vi "Test Helper - Echo Server.vi"(6 "Delay 1st reply only":bool, 7 "idle timout":u32=2000, 8 "Answer?":bool, 9 "reply delay (ms)":u32, 10 "number of messages":i32=1, 11 "port":u16=55501) -> (0 "error out":errorcluster, 2 "Commands":string[](array[string]))   [LabVIEW 2019, in "RemoteControl.ZMQ.Tests.lvclass"]
uses:
  RemoteControl.ZMQ.Tests.lvclass
panel:
  out "Numeric":i32
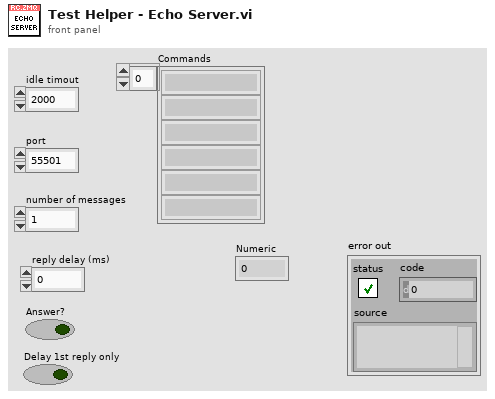
[diagram p1: front panel]
types:
  T1 = typedef "RemoteControl.lvlib/RemoteControl.lvclass/Message--Cluster.ctl" = cluster{"Command":string, "Data":variant, "ID":string, "error":errorcluster}
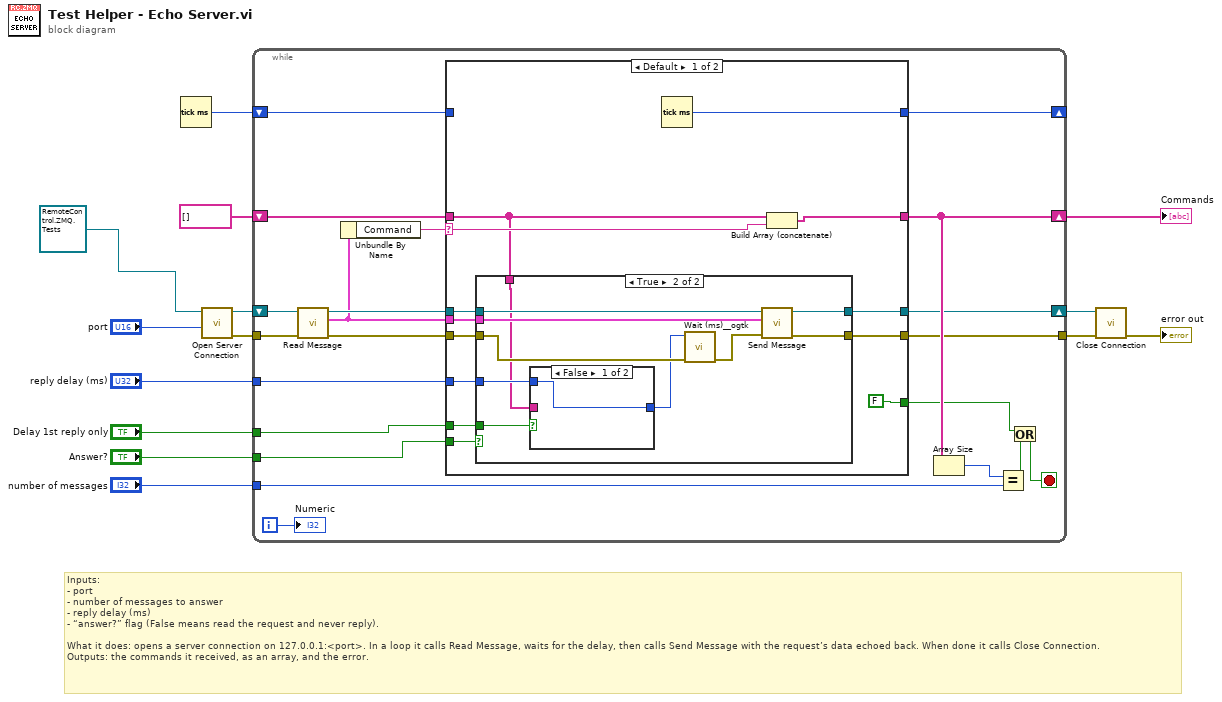
[diagram p0: block diagram]
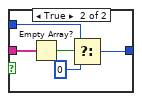
[diagram p3: hidden frame]
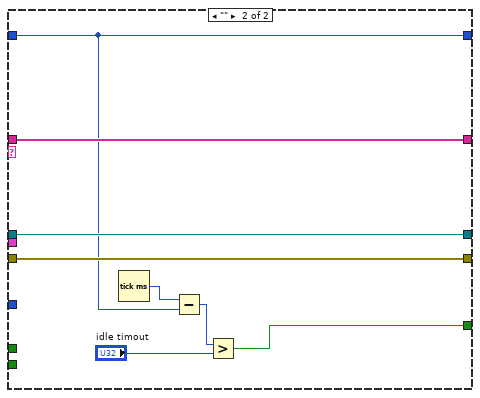
[diagram p4: hidden frame]
diagram:
  # "Inputs:\n- port\n- number of messages to answer\n- reply delay (ms)\n- “answer?” flag (False means read the request and never reply).\n\nWhat it does: opens a server connection on 127.0.0.1:<port>. In a loop it calls Read Message, waits for the delay, then calls Send Message with the request’s data echoed back. When done it calls Close Connection.\nOutputs: the commands it received, as an array, and the error."
  n1 = Tick Count (ms)() -> (millisecond timer value=w2:u32)
  n2 = call-dynamic "Open Server Connection.vi"("port"="port", "RemoteControl.ZMQ in"=refnum<class "RemoteControl.ZMQ.Tests.lvclass"> refnum ("RemoteControl.ZMQ.Tests.lvclass")) -> ("error out"=w12:errorcluster, "RemoteControl.ZMQ out"=w14:refnum<class "RemoteControl.ZMQ.Tests.lvclass">)  [unwired: 8 in]
  n3 = while {
    tunnel: "reply delay (ms)" -> [w18]
    tunnel: w12 -> [w34]
    tunnel: [w25] -> w11
    tunnel: "Answer?" -> [w26]
    tunnel: "number of messages" -> [w33]
    shift-right: [w28] -> w5
    shift-left: string[] [] -> [w30]
    tunnel: "Delay 1st reply only" -> [w19]
    shift-right: [w16] -> _
    shift-left: w2 -> [w15]
    shift-right: [w24] -> w10
    shift-left: w14 -> [w35]
    i -> [w29]
    stop <- w21 stop-if-true
    n4 = call-dynamic "Read Message.vi"("error in (no error)"=w34, "RemoteControl.ZMQ in"=w35) -> ("error out"=w20:errorcluster, "Message"=w17:T1, "RemoteControl.ZMQ out"=w27:refnum<class "RemoteControl.ZMQ.Tests.lvclass">)  [unwired: 7 in]
    n5 = Unbundle By Name(w17) -> ("Command"=w31:string)
    n6 = case shown="Default" w31 {
      selector: w31 -> [w48 _]
      tunnel: [w47 w74] -> w28
      tunnel: w30 -> [w39 w74]
      tunnel: w27 -> [w46 w73]
      tunnel: w26 -> [w45 _]
      tunnel: [w44 w72] -> w25
      tunnel: [w43 w73] -> w24
      tunnel: w17 -> [w42 _]
      tunnel: [FALSE ("x") w67] -> w23
      tunnel: w20 -> [w40 w72]
      tunnel: w19 -> [w38 _]
      tunnel: w18 -> [w37 _]
      tunnel: [w36 w70] -> w16
      tunnel: w15 -> [_ w70]
      frame Default {
        n7 = case shown="True" w45 {
          tunnel: w46 -> [w50 w60]
          tunnel: [w49 w59] -> w44
          tunnel: [w50 w58] -> w43
          tunnel: w42 -> [_ w57]
          tunnel: w40 -> [w49 w55]
          tunnel: w39 -> [_ w52]
          tunnel: w38 -> [_ w51]
          tunnel: w37 -> [_ w54]
          frame False {
          }
          frame True {
            n8 = case shown="False" w51 {
              tunnel: w54 -> [w61 w66]
              tunnel: [w61 w65] -> w53
              tunnel: w52 -> [_ w63]
              frame False {
              }
              frame True {
                n9 = Empty Array?(array=w63) -> (empty?=w62:bool)
                n10 = Select(t=w66, s=w62, f=u32 0) -> (s? t:f=w65:u32)
              }
            }
            n11 = call <userlib>:"Wait (ms)__ogtk.vi"("error in (no error)"=w55, "milliseconds to wait"=w53) -> ("error out"=w56:errorcluster)  [unwired: 8 in, 1 out]
            n12 = call-dynamic "Send Message.vi"("error in (no error)"=w56, "Message"=w57, "RemoteControl.ZMQ in"=w60) -> ("error out"=w59:errorcluster, "RemoteControl.ZMQ out"=w58:refnum<class "RemoteControl.ZMQ.Tests.lvclass">)  [unwired: 7 in]
          }
        }
        n13 = Tick Count (ms)() -> (millisecond timer value=w36:u32)
        n14 = Build Array (concatenate)(w39, w48) -> (w47:string[])
      }
      frame "" {
        n15 = Tick Count (ms)() -> (millisecond timer value=w71:u32)
        n16 = Subtract(x=w71, y=w70) -> (x-y=w69:u32)
        n17 = Greater?(x=w69, y="idle timout") -> (0:w67:bool)
      }
    }
    n18 = Array Size(array=w28) -> (size(s)=w32:i32)
    n19 = Equal?(x=w32, y=w33) -> (x = y?=w22:bool)
    n20 = Or(x=w23, y=w22) -> (x .or. y?=w21:bool)
    "Numeric" <- w29
  }
  "Commands" <- w5
  n21 = call-dynamic "Close Connection.vi"("error in (no error)"=w11, "RemoteControl.ZMQ in"=w10) -> ("error out"=→"error out":errorcluster)  [unwired: 8 in, 1 out]
